vi "SMTP Email Reply To Error.vi"(4 "error in (no error)":errorcluster caption="entrée d'erreur (pas d'erreur)", 5 "reply string in":string caption="chaîne de réponse en entrée", 6 "reply code in":i32 caption="code de réponse en entrée", 7 "smtp session":T1 caption="session smtp") -> (0 "error out":errorcluster caption="sortie d'erreur", 1 "duplicate reply string":string caption="chaîne de réponse dupliquée", 2 "duplicate reply code":i32 caption="code de réponse dupliqué", 3 "smtp session out":T1 caption="session smtp en sortie")   [LabVIEW 2022 SP3, in "Copie de NI_SMTPEmail.lvlib"]
doc: "Analyse les trois premiers chiffres d'une chaîne de réponse d'un serveur SMTP et définit la condition d'erreur du cluster \"sortie d'erreur\" à VRAI si le code d'erreur est supérieur à 400. En cas d'erreur, il définit aussi le code d'erreur du cluster au code d'erreur analysé, et le champ source à la chaîne de réponse (sans le code d'erreur)."
uses:
  Copie de NI_SMTPEmail.lvlib
  SMTP Email Session.ctl
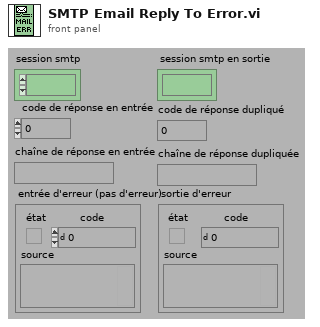
[diagram p1: front panel]
types:
  T1 = typedef "Copie de NI_SMTPEmail.lvlib/SMTP Email Session.ctl" = refnum<k1>
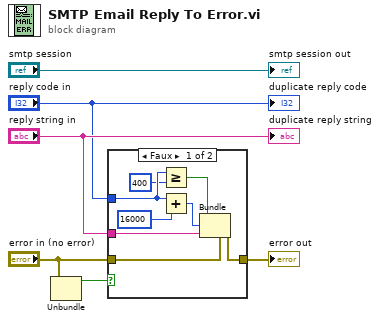
[diagram p0: block diagram]
diagram:
  n1 = Unbundle("error in (no error)") -> ("status"=w1:bool)  [unwired: 2 out]
  n2 = case shown="Faux" w1 {
    tunnel: "reply code in" -> [w14 _]
    tunnel: [w13 w15] -> w4
    tunnel: "reply string in" -> [w10 _]
    tunnel: "error in (no error)" -> [w9 w15]
    frame False {
      n3 = Greater Or Equal?(x=w14, y=400) -> (x >= y?=w8:bool)
      n4 = Add(x=w14, y=16000) -> (x+y=w12:i32)
      n5 = Bundle(cluster=w9, "status"=w8, "code"=w12, "source"=w10) -> (w13:errorcluster)
    }
    frame True {
    }
  }
  "error out" <- w4
  "duplicate reply code" <- "reply code in"
  "duplicate reply string" <- "reply string in"
  "smtp session out" <- "smtp session"
